vi "type.set.vi"(8 "error in":errorcluster, 10 "type":refnum<class "type.lvclass">, 11 "asset in":refnum<class "asset.lvclass">) -> (0 "error out":errorcluster, 3 "asset out":refnum<class "asset.lvclass">)   [LabVIEW 2020, in "asset.lvclass"]
uses:
  asset.lvclass
  type/type.lvclass
  asset.lvclass/asset.ctl
  type/type.lvclass/type.ctl
  Nominal Client/Nominal Client.lvclass/Nominal Client.ctl
  type/rid.get.vi
  Nominal Client/error.vi
  Nominal Client/trace.payload_sent.vi
  Nominal Client/trace.payload_received.vi
  Nominal Client/create.authorization_header.vi
  Nominal Client/error.vi/859f8e04-e495-489b-b5b4-7ac163f56130.vi
  Nominal Client/trace.generate.vi
  <vilib>/AdvancedString/1D String Array to Delimited String.vi
  <vilib>/JDP Science/JDP Science Common Utilities/Trim Whitespace__JDP.vi
  Nominal Client/trace.calling_method.vi
  Nominal Client/api_token.get.vi
  <vilib>/Utility/libraryn.llb/Get File Extension.vi
  Nominal Client/log_file.write.vi
  <vilib>/JDP Science/JSONtext/Get all Object Items.vi
  <vilib>/Utility/error.llb/Error Cluster From Error Code.vi
  <vilib>/JDP Science/JSONtext/JSON text to Variant.vi
  <vilib>/JDP Science/JSONtext/LVClass Serializer/JSONtext LVClass Serializer.lvclass
  <vilib>/addons/_JKI.lib/REST Client/classes/Response Headers/Response Headers.lvclass
  <vilib>/addons/_JKI.lib/REST Client/classes/REST Client/REST Client.lvclass
  Nominal Client/Nominal Client.lvclass
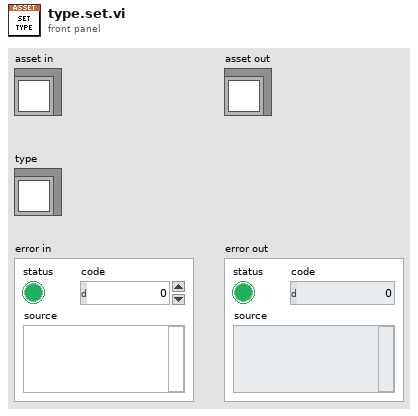
[diagram p1: front panel]
types:
  T1 = typedef "dataScopes.lvlib/links.ctl" = cluster{"URL":string, "Title":string}[]
  T2 = typedef "dataScopes.lvlib/data_scopes.ctl" = T3[]
  T3 = typedef "dataScopes.lvlib/data_scope.ctl" = cluster{"dataScopeName":string, "dataSource":T4, "seriesTags":refnum<class "properties.lvclass">, "offset":T6}
  T4 = typedef "dataScopes.lvlib/data_source.ctl" = cluster{"type":T5, "rid":string}
  T5 = typedef "dataScopes.lvlib/type.ctl" = enum16{"dataset", "connection", "logSet", "video"}
  T6 = typedef "dataScopes.lvlib/offset.ctl" = cluster{"seconds":i32, "nanos":i32, "picos":i32}
  T7 = cluster{"rid":string, "title":string, "properties":refnum<class "properties.lvclass">, "labels":refnum<class "labels.lvclass">, "Links":T1, "datascopes":T2, "createdAt":timestamp, "updatedAt":timestamp, "attachments":refnum<class "labels.lvclass">, "isStaged":bool, "isArchived":bool, "description":string, "createdBy":string, "type":string}
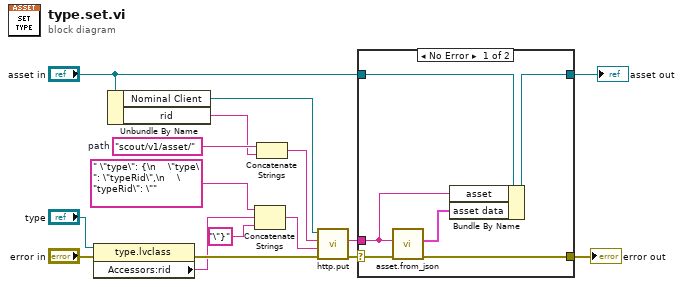
[diagram p0: block diagram]
diagram:
  w15 = "scout/v1/asset/"  # path
  n1 = property class="type.lvclass"(reference="type", error in="error in") -> (error out=w3:errorcluster, "Accessors:rid"=w1:string)  [unwired: 1 out]
  n2 = Unbundle By Name("asset in") -> ("Nominal Client"=w16:refnum<class "Nominal Client.lvclass">, "rid"=w13:string)
  n3 = Concatenate Strings(" \"type\": {\n    \"type\": \"typeRid\",\n    \"typeRid\": \"", w1, "\"}") -> (w6:string)
  n4 = Concatenate Strings(w15, w13) -> (w14:string)
  n5 = call "http.put.vi"("error in"=w3, "Body"=w6, "Path"=w14, "Nominal Client in"=w16) -> ("error out"=w12:errorcluster, "Response"=w9:string)  [unwired: 4 in, 2 out]
  n6 = case shown="No Error" w12 {
    selector: w12 -> [w22 w24]
    tunnel: [w21 w24] -> w11
    tunnel: "asset in" -> [w20 w23]
    tunnel: w9 -> [w18 _]
    tunnel: [w17 w23] -> w8
    frame No Error {
      n7 = call "asset.from_json.vi"("error in"=w22, "asset"=w18) -> ("error out"=w21:errorcluster, "Asset Data"=w19:T7)  [unwired: 8 in]
      n8 = Bundle By Name(cluster=w20, "asset"=w18, "asset data"=w19) -> (w17:refnum<class "asset.lvclass">)
    }
    frame Error {
    }
  }
  "asset out" <- w8
  "error out" <- w11
